vi "Scale Params.vi"(7 "SensorList (Auto)":refnum<class "SensorList.lvclass">, 8 "error in (no error)":errorcluster, 11 "Scale in":refnum<class "Scale Config.lvclass">) -> (0 "error out":errorcluster, 1 "Scale Params":dbl[](array[numeric]), 2 "Scale Type":T1, 3 "Scale out":refnum<class "Scale Config.lvclass">)   [LabVIEW 2020, in "VolatusConfig.lvlib" / "Scale Config.lvclass"]
uses:
  Scale Config.lvclass
  C:/dev/lv20CE/relink/lv-volatus/VolatusConfig/VolatusConfigElement/VolatusConfigElement.lvclass
  SensorList/SensorList.lvclass
  Scale Type.ctl
  VolatusConfigElement/VolatusConfigElement.lvclass/VolatusConfigElement.ctl
  VolatusConfigElement/Element.vi
  VolatusConfigElement/VolatusConfigElement.lvclass
  lv-cdm/CDM-Config/Config Element/Config Element.lvclass
  VolatusConfig.lvlib
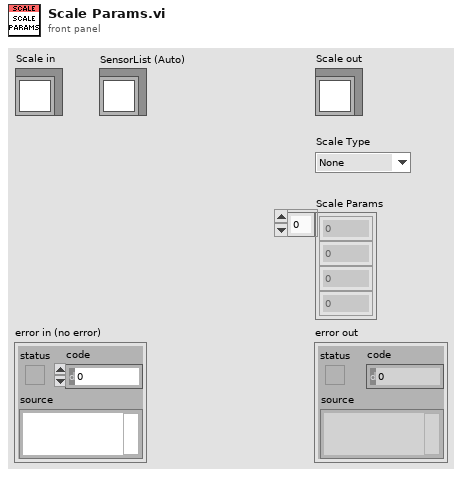
[diagram p1: front panel]
types:
  T1 = typedef "VolatusConfig.lvlib/Scale Type.ctl" = enum16{"None", "Sensor", "Polynomial", "Threshold", "Invert Bool", "Exponential"}
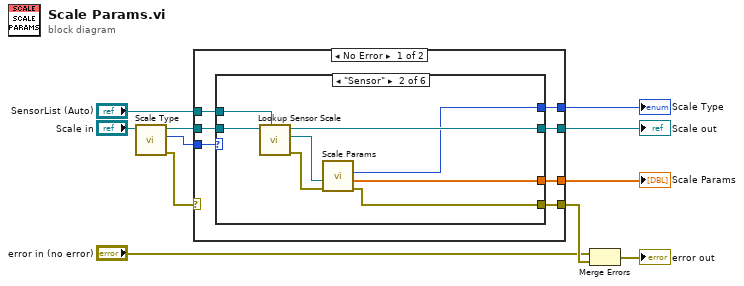
[diagram p0: block diagram]
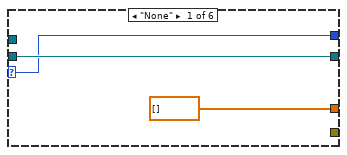
[diagram p2: hidden frame]
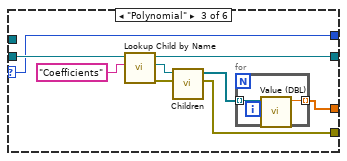
[diagram p3: hidden frame]
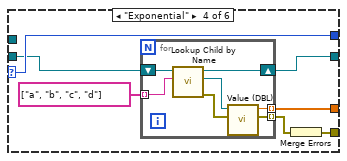
[diagram p4: hidden frame]
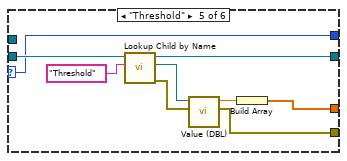
[diagram p5: hidden frame]
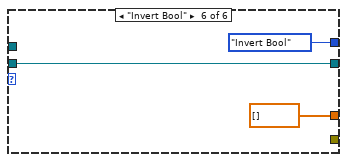
[diagram p6: hidden frame]
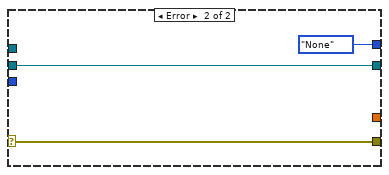
[diagram p7: hidden frame]
diagram:
  n1 = call "Scale Type.vi"("Scale in"="Scale in") -> ("error out"=w11:errorcluster, "Scale Type"=w2:T1, "Scale out"=w9:refnum<class "Scale Config.lvclass">)  [unwired: 8 in]
  n2 = case shown="No Error" w11 {
    selector: w11 -> [_ w69]
    tunnel: [w18 w69] -> w10
    tunnel: w9 -> [w17 w68]
    tunnel: [w16 w68] -> w7
    tunnel: [w15 _] -> w4
    tunnel: w2 -> [w14 _]
    tunnel: "SensorList (Auto)" -> [w13 _]
    tunnel: [w12 Scale_Type."None" ("Scale Type")] -> w1
    frame No Error {
      n3 = case shown="\"Sensor\"" w14 {
        selector: w14 -> [w19 _ w30 w46 w55 _]
        tunnel: [_ w26 w33 w41 w57 _] -> w18
        tunnel: w17 -> [w21 w29 w38 w45 w63 w65]
        tunnel: [w21 w28 w32 w43 w61 w65] -> w16
        tunnel: [dbl[] [] w24 w31 w47 w56 dbl[] [] ("Scale Params")] -> w15
        tunnel: w13 -> [_ w25 _ _ _ _]
        tunnel: [w19 w23 w30 w46 w55 Scale_Type."Invert Bool" ("Scale Type")] -> w12
        frame "None" {
        }
        frame "Sensor" {
          n4 = call "Lookup Sensor Scale.vi"("SensorList"=w25, "Scale in"=w29) -> ("error out"=w27:errorcluster, "Sensor Scale"=w22:refnum<class "Scale Config.lvclass">, "Scale out"=w28:refnum<class "Scale Config.lvclass">)  [unwired: 7 in]
          n5 = call "Scale Params.vi"("error in (no error)"=w27, "Scale in"=w22) -> ("error out"=w26:errorcluster, "Scale Params"=w24:dbl[], "Scale Type"=w23:T1)  [unwired: 6 in, 1 out]
        }
        frame "Polynomial" {
          n6 = call "Lookup Child by Name.vi"("Child Name"="Coefficients", "VolatusConfigElement in"=w38) -> ("error out"=w36:errorcluster, "Child"=w35:refnum<class "Config Element.lvclass">, "VolatusConfigElement out"=w32:refnum<class "Scale Config.lvclass">)  [unwired: 6 in, 1 out]
          n7 = call "Children.vi"("error in (no error)"=w36, "Config Element in"=w35) -> ("error out"=w33:errorcluster, "Elements"=w34:refnum<class "Config Element.lvclass">[])  [unwired: 8 in]
          n8 = for {
            tunnel: w34 -> [w40] mode=indexing
            tunnel: [w39] -> w31 mode=indexing
            n9 = call "Value (DBL).vi"("Config Element in"=w40) -> ("DBL Value"=w39:dbl)  [unwired: 9 in, 1 out]
          }
        }
        frame "Exponential" {
          n10 = for {
            tunnel: [w54] -> w47 mode=indexing
            shift-right: [w49] -> w43
            shift-left: w45 -> [w53]
            tunnel: string[] ["a", "b", "c", "d"] -> [w52] mode=indexing
            tunnel: [w48] -> w42 mode=indexing
            n11 = call "Lookup Child by Name.vi"("Child Name"=w52, "VolatusConfigElement in"=w53) -> ("error out"=w50:errorcluster, "Child"=w51:refnum<class "Config Element.lvclass">, "VolatusConfigElement out"=w49:refnum<class "Scale Config.lvclass">)  [unwired: 6 in, 1 out]
            n12 = call "Value (DBL).vi"("error in (no error)"=w50, "Config Element in"=w51) -> ("error out"=w48:errorcluster, "DBL Value"=w54:dbl)  [unwired: 8 in]
          }
          n13 = Merge Errors(w42) -> (w41:errorcluster)
        }
        frame "Threshold" {
          n14 = call "Lookup Child by Name.vi"("Child Name"="Threshold", "VolatusConfigElement in"=w63) -> ("error out"=w58:errorcluster, "Child"=w59:refnum<class "Config Element.lvclass">, "VolatusConfigElement out"=w61:refnum<class "Scale Config.lvclass">)  [unwired: 6 in, 1 out]
          n15 = call "Value (DBL).vi"("error in (no error)"=w58, "Config Element in"=w59) -> ("error out"=w57:errorcluster, "DBL Value"=w60:dbl)  [unwired: 8 in]
          n16 = Build Array(w60) -> (w56:dbl[])
        }
        frame "Invert Bool" {
        }
      }
    }
    frame Error {
    }
  }
  "Scale out" <- w7
  "Scale Params" <- w4
  "Scale Type" <- w1
  n17 = Merge Errors("error in (no error)", w10) -> (→"error out":errorcluster)
